vi "check Abort (ActiveJob).vi"(7 "Abort is Error? (F)":bool, 8 "error in (no error)":errorcluster, 9 "timeout (0 ms)":i32, 11 "Job in":refnum<class "Job.lvclass">) -> (0 "error out":errorcluster, 1 "exception":i32, 2 "Abort":bool, 3 "Job out":refnum<class "Job.lvclass">)   [LabVIEW 2013, in "openCronJob.lvlib" / "Job.lvclass"]
uses:
  Job.lvclass
  Job.lvclass/Job.ctl
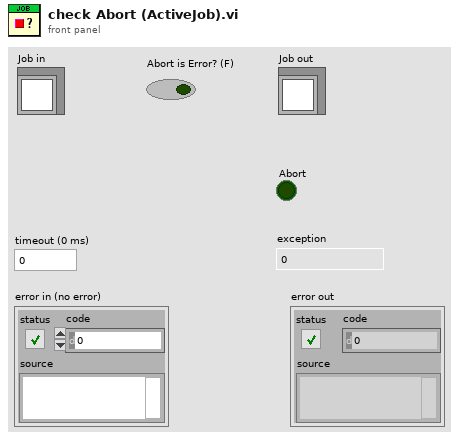
[diagram p1: front panel]
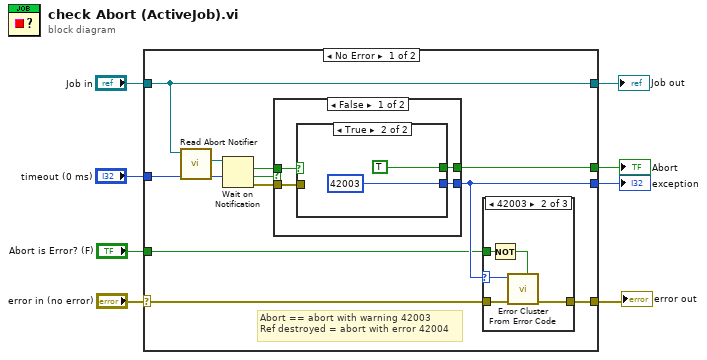
[diagram p0: block diagram]
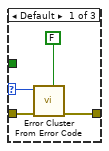
[diagram p2: hidden frame]
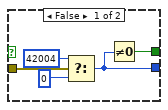
[diagram p4: hidden frame]
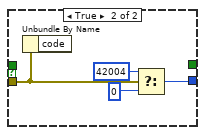
[diagram p5: hidden frame]
diagram:
  n1 = case shown="No Error" "error in (no error)" {
    selector: "error in (no error)" -> [w10 w46]
    tunnel: [w19 _] -> w8
    tunnel: [w12 _] -> w7
    tunnel: "timeout (0 ms)" -> [w16 _]
    tunnel: "Job in" -> [w13 w45]
    tunnel: [w13 w45] -> w3
    tunnel: [w11 w46] -> w2
    tunnel: "Abort is Error? (F)" -> [w9 _]
    frame No Error {
      # "Abort == abort with warning 42003\nRef destroyed = abort with error 42004"
      n2 = call "Read Abort Notifier.vi"("Job in"=w13) -> ("Abort"=w15:refnum<notifier>)  [unwired: 10 in]
      n3 = Wait on Notification(notifier=w15, timeout in ms (-1)=w16) -> (notification=w17:bool, timed out?=w14:bool, error out=w18:errorcluster)  [unwired: 2 in, 1 out]
      n4 = case shown="False" w14 {
        tunnel: [w33 _] -> w19
        tunnel: w18 -> [w32 w41]
        tunnel: w17 -> [w31 _]
        tunnel: [w30 w42] -> w12
        frame False {
          n5 = case shown="True" w31 {
            tunnel: [w34 42003 ("exception")] -> w30
            tunnel: w32 -> [w38 _]
            tunnel: [w35 TRUE] -> w33
            frame False {
              n6 = Select(t=42004, s=w38, f=0 ("exception")) -> (s? t:f=w34:i32)
              n7 = Not Equal To 0?(x=w34) -> (x != 0?=w35:bool)
            }
            frame True {
            }
          }
        }
        frame True {
          n8 = Unbundle By Name(w41) -> ()  [unwired: 1 out]
          n9 = Select(t=42004, s=w41, f=0 ("exception")) -> (s? t:f=w42:i32)
        }
      }
      n10 = case shown="42003" w12 {
        selector: w12 -> [w21 w26 _]
        tunnel: [w22 w27 w29] -> w11
        tunnel: w10 -> [w23 w28 w29]
        tunnel: w9 -> [_ w25 _]
        frame Default {
          n11 = call <vilib>:"Error Cluster From Error Code.vi"("is warning? (False)"=FALSE, "error in (no error)"=w23, "error code (0)"=w21) -> ("error out"=w22:errorcluster)  [unwired: 6 in]
        }
        frame 42003 {
          n12 = Not(x=w25) -> (.not. x?=w24:bool)
          n13 = call <vilib>:"Error Cluster From Error Code.vi"("is warning? (False)"=w24, "error in (no error)"=w28, "error code (0)"=w26) -> ("error out"=w27:errorcluster)  [unwired: 6 in]
        }
        frame 0 {
        }
      }
    }
    frame Error {
    }
  }
  "Abort" <- w8
  "exception" <- w7
  "Job out" <- w3
  "error out" <- w2
